vi "Func - Unflatten Error Handler (Error Cluster).vi"(7 "InstanceRef":T1, 8 "Unflatten Error Cluster":errorcluster, 9 "error status before":bool, 10 "argument number":i32=-1, 11 "name":string) -> (0 "Error Cluster out":errorcluster, 1 "error status out":bool, 3 "dup name":string)   [LabVIEW 2021]
doc: "This VI handles an error produced by the <b>Unflatten From String</b> LabVIEW function. Refer to the VI help for more details.\n\n<b>name</b> is ignored and passed directly to <b>dup name</b>.\n\n<b>argument number</b> control specifies the argument number where an unflattening error occurs. The VI adds the argument number to the error description to simplify debugging.\n\n<b>error status before</b> control is used to indicate an error occurred before calling the Unflatten From String function to avoid irrelevant error messages from being added to the CE Error Log.\n\n<b>Unflatten Error Cluster</b> control must be connected to the <b>error out</b> terminal of the Unflatten From String</b> LabVIEW function.\n\n::: CalcExpress Toolkit :::\nCopyright (c) 2000-2026 Konstantin Shifershteyn. All rights reserved."
uses:
  cetypes.llb/CalcExpress Instance RefNum.ctl
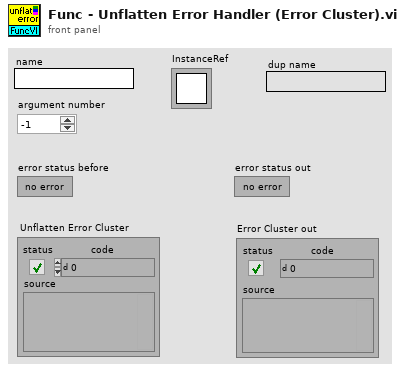
[diagram p1: front panel]
types:
  T1 = typedef "CalcExpress Instance RefNum.ctl" = refnum<k1>
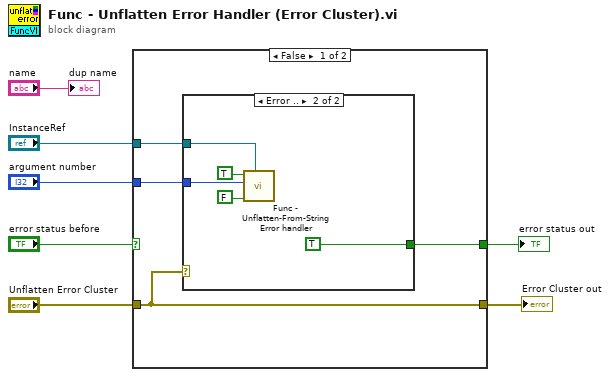
[diagram p0: block diagram]
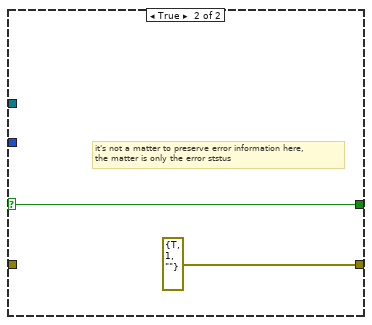
[diagram p3: hidden frame]
diagram:
  n1 = case shown="False" "error status before" {
    selector: "error status before" -> [_ w17]
    tunnel: "Unflatten Error Cluster" -> [w11 _]
    tunnel: [w11 errorcluster {"status"=TRUE, "code"=1, "source"=""} ("error constant")] -> w5
    tunnel: "argument number" -> [w10 _]
    tunnel: "InstanceRef" -> [w9 _]
    tunnel: [w8 w17] -> w1
    frame False {
      n2 = case shown="Error .." w11 {
        tunnel: w10 -> [_ w16]
        tunnel: w9 -> [_ w15]
        tunnel: [_ TRUE] -> w8
        frame No Error {
        }
        frame Error {
          n3 = call "Func - Unflatten-From-String Error handler.vi"("InstanceRef"=w15, "error in"=FALSE, "argument number"=w16, "Unflatten Error status"=TRUE) -> ()  [unwired: 5 in, 1 out]
        }
      }
    }
    frame True {
      # "it's not a matter to preserve error information here,\nthe matter is only the error ststus"
    }
  }
  "Error Cluster out" <- w5
  "error status out" <- w1
  "dup name" <- "name"
